vi "io_refnum.vi"(11 "ivi":refnum<k15>) -> ()   [LabVIEW 2020]
panel:
  in  "sv":refnum<k21>
  in  "visa":refnum<visa-resource-name>
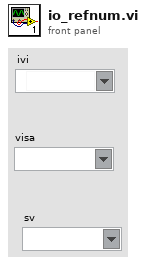
[diagram p1: front panel]
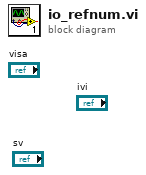
[diagram p0: block diagram]
diagram:
